vi "Filter.vi"(10 "file path":path, 11 "CleanupFilter.LastMod in":refnum<class "CleanupFilter.LastMod.lvclass">) -> (2 "cleanup?":bool, 3 "CleanupFilter.LastMod out":refnum<class "CleanupFilter.LastMod.lvclass">)   [LabVIEW 2018, in "GLog.lvlib" / "CleanupFilter.LastMod.lvclass"]
uses:
  CleanupFilter.LastMod.lvclass
  CleanupFilter.LastMod.lvclass/CleanupFilter.LastMod.ctl
panel:
  # "Connector Pane"
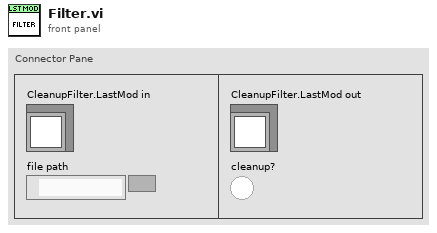
[diagram p1: front panel]
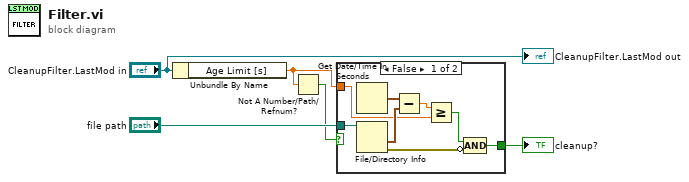
[diagram p0: block diagram]
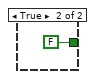
[diagram p2: hidden frame]
diagram:
  n1 = Unbundle By Name("CleanupFilter.LastMod in") -> ("Age Limit [s]"=w1:dbl)
  n2 = Not A Number/Path/Refnum?(number/path/refnum=w1) -> (NaN/Path/Refnum?=w2:bool)
  n3 = case shown="False" w2 {
    tunnel: "file path" -> [w10 _]
    tunnel: [w7 FALSE] -> w4
    tunnel: w1 -> [w8 _]
    frame False {
      n4 = Get Date/Time In Seconds() -> (seconds since 1Jan1904=w12:timestamp)
      n5 = File/Directory Info(path=w10) -> (last mod=w13:timestamp, error out=w6:errorcluster)  [unwired: 1 in, 5 out]
      n6 = Subtract(x=w12, y=w13) -> (x-y=w11:dbl)
      n7 = Greater Or Equal?(x=w11, y=w8) -> (x >= y?=w9:bool)
      n8 = Compound Arithmetic op=AND(w9, invert w6) -> (w7:bool)
    }
    frame True {
    }
  }
  "cleanup?" <- w4
  "CleanupFilter.LastMod out" <- "CleanupFilter.LastMod in"
